vi "Test Shuffle Array.vi"() -> ()   [LabVIEW 2012]
uses:
  Shuffle Array.xnode
panel:
  out "Shuffled Array":string[](array[string])
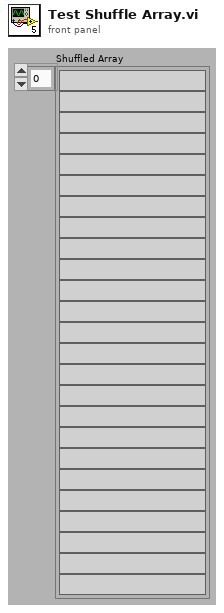
[diagram p1: front panel]
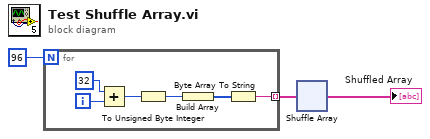
[diagram p0: block diagram]
diagram:
  n1 = for {
    N: 96 -> [_]
    tunnel: [w4] -> w1 mode=indexing
    i -> [w9]
    n2 = Add(x=32, y=w9) -> (x+y=w7:i32)
    n3 = To Unsigned Byte Integer(number=w7) -> (unsigned 8bit integer=w6:u8)
    n4 = Build Array(w6) -> (w5:u8[])
    n5 = Byte Array To String(unsigned byte array=w5) -> (string=w4:string)
  }
  n6 = xnode "Shuffle Array"("Array In"=w1) -> ("Shuffled Array"=→"Shuffled Array":string[])
